vi "eDyno Speed Profile.vi"(0 "Speed Profile":T1={"Run-up Enabled"=FALSE, "Constant Speed (rpm)"=3000.0, "Run-up Start (rpm)"=500.0, "Run-up End (rpm)"=4500.0, "Run-up Duration (s)"=30.0}, 5 "t in (s)":dbl, 7 "Block Duration (s)":dbl=0.1) -> (4 "rpm start":dbl, 6 "rpm end":dbl, 8 "t out (s)":dbl)   [LabVIEW 2026]
doc: "Speed for the next block. Constant: rpm start = rpm end = Constant Speed. Run-up (Run-up Enabled ON): linear ramp from Run-up Start to Run-up End over Run-up Duration, then holds at Run-up End. Elapsed run-up time travels in t in / t out (keep it in a shift register in the caller); it resets to 0 whenever Run-up Enabled is OFF, so switching it ON restarts the run-up."
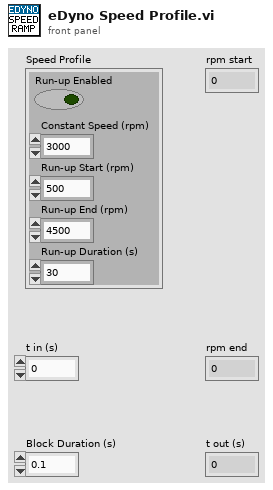
[diagram p1: front panel]
types:
  T1 = cluster{"Run-up Enabled":bool, "Constant Speed (rpm)":dbl, "Run-up Start (rpm)":dbl, "Run-up End (rpm)":dbl, "Run-up Duration (s)":dbl}
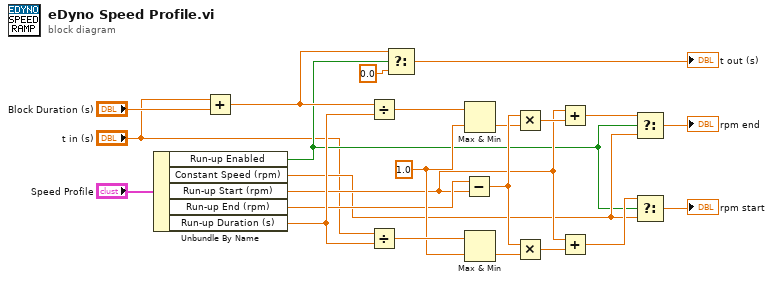
[diagram p0: block diagram]
diagram:
  w14 = 1.0 ("one")
  n1 = Unbundle By Name("Speed Profile") -> ("Run-up Enabled"=w7:bool, "Constant Speed (rpm)"=w8:dbl, "Run-up Start (rpm)"=w9:dbl, "Run-up End (rpm)"=w10:dbl, "Run-up Duration (s)"=w11:dbl)
  n2 = Add(x="t in (s)", y="Block Duration (s)") -> (x+y=w12:dbl)
  n3 = Divide(x=w12, y=w11) -> (x/y=w17:dbl)
  n4 = Divide(x="t in (s)", y=w11) -> (x/y=w15:dbl)
  n5 = Select(t=w12, s=w7, f=0.0 ("zero")) -> (s? t:f=→"t out (s)":dbl)
  n6 = Subtract(x=w10, y=w9) -> (x-y=w19:dbl)
  n7 = Max & Min(x=w17, y=w14) -> (min(x,y)=w18:dbl)  [unwired: 1 out]
  n8 = Max & Min(x=w15, y=w14) -> (min(x,y)=w16:dbl)  [unwired: 1 out]
  n9 = Multiply(x=w19, y=w18) -> (x*y=w22:dbl)
  n10 = Multiply(x=w19, y=w16) -> (x*y=w20:dbl)
  n11 = Add(x=w9, y=w22) -> (x+y=w23:dbl)
  n12 = Add(x=w9, y=w20) -> (x+y=w21:dbl)
  n13 = Select(t=w23, s=w7, f=w8) -> (s? t:f=→"rpm end":dbl)
  n14 = Select(t=w21, s=w7, f=w8) -> (s? t:f=→"rpm start":dbl)
